vi "resize_cubic_planar.vi"(8 "error in (no error)":errorcluster, 9 "target_h":i32=1024, 10 "target_w":i32=1024, 11 "image in":T1) -> (0 "error out":errorcluster, 3 "image out":T1)   [LabVIEW 2017, in "Image Processing Library.lvlib"]
uses:
  Image Processing Library.lvlib
  <vilib>/picture/picture.llb/imagedata.ctl
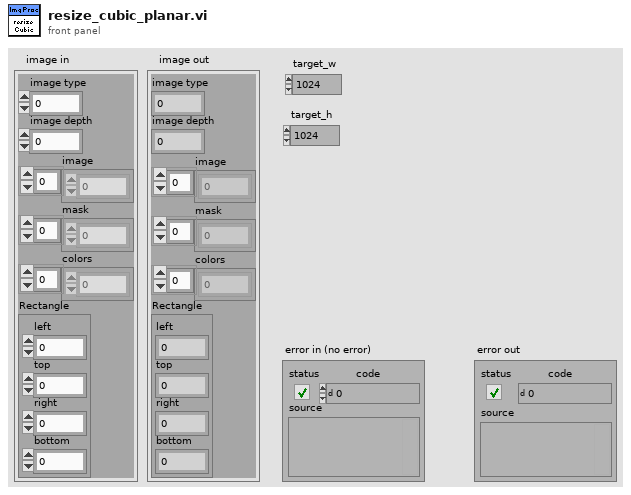
[diagram p1: front panel]
types:
  T1 = typedef "imagedata.ctl" = cluster{"image type":i32, "image depth":i32, "image":u8[], "mask":u8[], "colors":u32[], "Rectangle":cluster{"left":i16, "top":i16, "right":i16, "bottom":i16}}
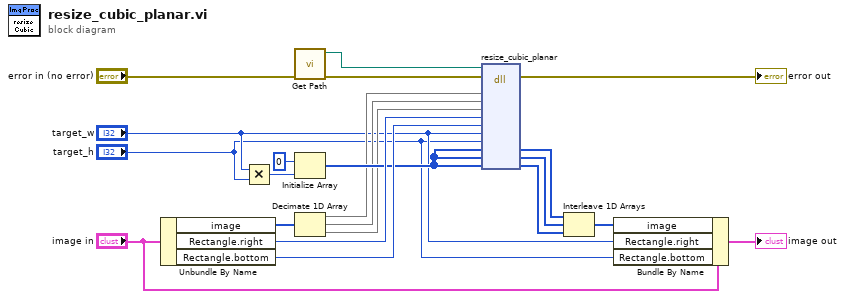
[diagram p0: block diagram]
diagram:
  n1 = Unbundle By Name("image in") -> ("image"=w12:u8[], "Rectangle.right"=w17:i16, "Rectangle.bottom"=w16:i16)
  n2 = Multiply(x="target_w", y="target_h") -> (x*y=w15:i32)
  n3 = call "Get Path.vi"("error in (no error)"="error in (no error)") -> ("error out"=w20:errorcluster, "Library Path"=w19:path)  [unwired: 9 in]
  n4 = Initialize Array(u8 0 ("element"), w15) -> (w13:u8[])
  n5 = Decimate 1D Array(w12) -> (w11:u8[], w10:u8[], w9:u8[])
  n6 = dll-call lib="C:/Users/IvanLis-Win10/Desktop/LabVIEW/Coin Detector/Project_2018/image_processing/windows_x64/image_processing.dll" fn="resize_cubic_planar"(path in=w19, error in=w20, "in_r"=w11, "in_g"=w10, "in_b"=w9, "orig_w"=w17, "orig_h"=w16, "target_w"="target_w", "target_h"="target_h", "out_r"=w13, "out_g"=w13, "out_b"=w13) -> (error out=→"error out":errorcluster, "out_r"=w8:u8[], "out_g"=w7:u8[], "out_b"=w6:u8[])  [unwired: 9 in, 1 out]
  n7 = Interleave 1D Arrays(w8, w7, w6) -> (w5:u8[])
  n8 = Bundle By Name(cluster="image in", "image"=w5, "Rectangle.right"="target_w", "Rectangle.bottom"="target_h") -> (→"image out":T1)
